vi "set Sweep Time.vi"(8 "error in (no error)":errorcluster, 9 "Sweep Time Auto?":bool, 10 "Sweep Time(sec)":dbl, 11 "Keysight 9020A in":refnum<class "Keysight 9020A.lvclass">) -> (0 "error out":errorcluster, 3 "Keysight 9020A out":refnum<class "Keysight 9020A.lvclass">)   [LabVIEW 2023, in "Spectrum Analyzer.lvlib" / "Keysight 9020A.lvclass"]
uses:
  Keysight 9020A.lvclass
  Keysight 9020A.lvclass/Keysight 9020A.ctl
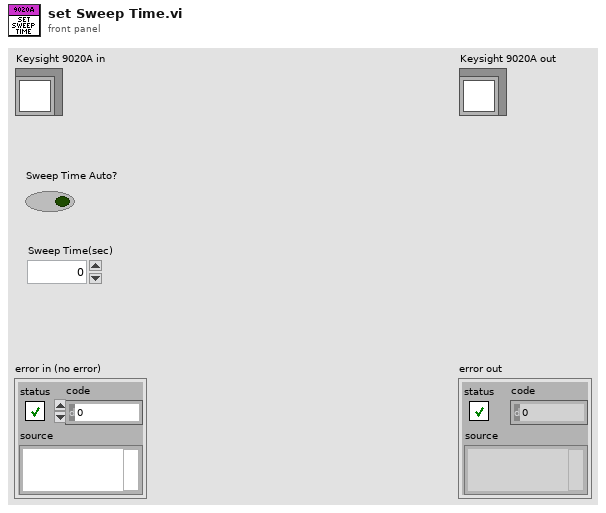
[diagram p1: front panel]
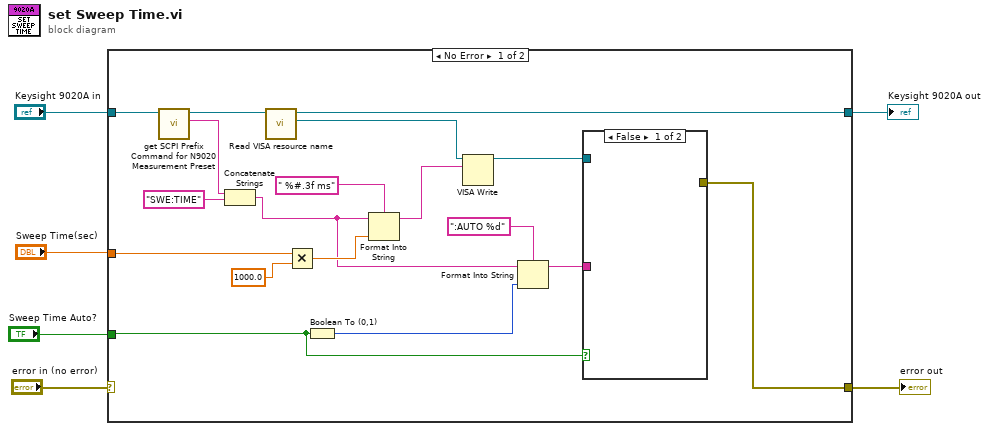
[diagram p0: block diagram]
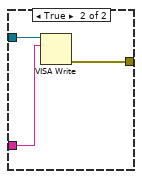
[diagram p2: hidden frame]
diagram:
  n1 = case shown="No Error" "error in (no error)" {
    selector: "error in (no error)" -> [_ w28]
    tunnel: "Keysight 9020A in" -> [w13 w29]
    tunnel: [w24 w29] -> w5
    tunnel: [w8 w28] -> w2
    tunnel: "Sweep Time(sec)" -> [w22 _]
    tunnel: "Sweep Time Auto?" -> [w7 _]
    frame No Error {
      n2 = call "get SCPI Prefix Command for N9020 Measurement Preset.vi"("Keysight 9020A in"=w13) -> ("SCPI Prefix Command"=w10:string, "Keysight 9020A out"=w12:refnum<class "Keysight 9020A.lvclass">)  [unwired: 8 in, 1 out]
      n3 = Concatenate Strings(w10, "SWE:TIME") -> (w9:string)
      n4 = call "Read VISA resource name.vi"("Keysight 9020A in"=w12) -> ("VISA resource name"=w14:refnum<visa-resource-name>, "Keysight 9020A out"=w24:refnum<class "Keysight 9020A.lvclass">)  [unwired: 8 in, 1 out]
      n5 = Multiply(x=w22, y=1000.0) -> (x*y=w20:dbl)
      n6 = Boolean To (0,1)(Boolean=w7) -> (0, 1=w15:i16)
      n7 = Format Into String(format string=" %#.3f ms", initial string=w9, w20) -> (resulting string=w23:string)  [unwired: 1 in, 1 out]
      n8 = VISA Write(VISA resource name=w14, write buffer=w23) -> (VISA resource name out=w18:refnum<visa-resource-name>)  [unwired: 1 in, 2 out]
      n9 = Format Into String(format string=":AUTO %d", initial string=w9, w15) -> (resulting string=w16:string)  [unwired: 1 in, 1 out]
      n10 = case shown="False" w7 {
        tunnel: w18 -> [_ w27]
        tunnel: w16 -> [_ w26]
        tunnel: [_ w25] -> w8
        frame False {
        }
        frame True {
          n11 = VISA Write(VISA resource name=w27, write buffer=w26) -> (error out=w25:errorcluster)  [unwired: 1 in, 2 out]
        }
      }
    }
    frame Error {
    }
  }
  "error out" <- w2
  "Keysight 9020A out" <- w5
